vi "I2C Open.vi"(8 "error in (no error)":errorcluster, 11 "Slave Id":u8) -> (0 "error out":errorcluster, 3 "I2C Device out":T1)   [LabVIEW 2020, in "wiringPi.lvlib"]
doc: "<b>_______________________________________________________________</b>\n** Author: Juan José Villacorta\n** LabVIEW wrapper for C library <b> wiringPi </b>,\n** https://github.com/WiringPi/WiringPi\n<b>_______________________________________________________________</b>\n/*\n * Opens an I2C slave device \n**********************************************************************************\n*/"
uses:
  wiringPi.lvlib
  Type Defs/I2C Device.ctl
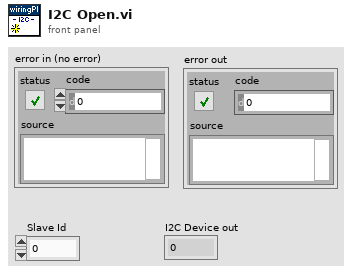
[diagram p1: front panel]
types:
  T1 = typedef "wiringPi.lvlib/I2C Device.ctl" = i32
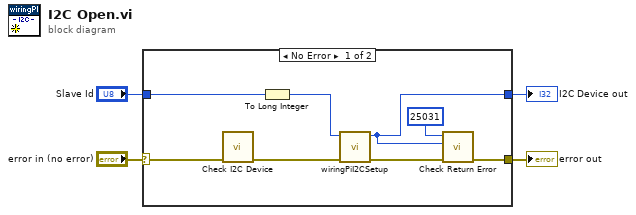
[diagram p0: block diagram]
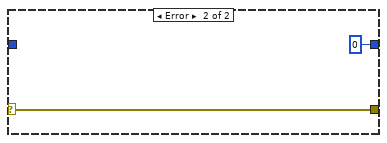
[diagram p2: hidden frame]
diagram:
  n1 = case shown="No Error" "error in (no error)" {
    selector: "error in (no error)" -> [w10 w14]
    tunnel: [w12 w14] -> w3
    tunnel: "Slave Id" -> [w6 _]
    tunnel: [w7 0 ("return")] -> w1
    frame No Error {
      n2 = call "Check I2C Device.vi"("error in (no error)"=w10) -> ("error out"=w9:errorcluster)  [unwired: 10 in]
      n3 = To Long Integer(number=w6) -> (32bit integer=w5:i32)
      n4 = call "wiringPiI2CSetup.vi"("error in (no error)"=w9, "devID"=w5) -> ("error out"=w8:errorcluster, "return"=w7:T1)  [unwired: 8 in]
      n5 = call "Check Return Error.vi"("error in (no error)"=w8, "Return code"=w7, "Error number"=25031) -> ("error out"=w12:errorcluster)  [unwired: 8 in]
    }
    frame Error {
    }
  }
  "error out" <- w3
  "I2C Device out" <- w1
